vi "Angle Alignment.vi"(9 "IMU Reading":dbl, 10 "Setpoint":dbl) -> (1 "Finished":bool, 2 "output":dbl format="%.2f")   [LabVIEW 2025]
doc: "Heading controller used by the Drive Controller \"Turn Aligning\" mode (structure from Reefscape 2025). Setpoint and IMU Reading are yaw in degrees (rounded to whole degrees). Outside +/- IMU Tolerance it runs a Parallel PID and returns the motor output; inside tolerance output is 0. Default gains: Everybot-tuned P and D (Kp 0.01, Kd 0.0006) plus the Reefscape integral (Ki 0.01), output +/-0.5. Finished is true once the heading is within tolerance AND the robot has settled: Pigeon accelerometer X magnitude < 350 and yaw rate (Pigeon raw gyro Z) magnitude < 5 deg/s."
uses:
  <vilib>/Rock Robotics/WPI/ThirdParty/Phoenix-LabVIEW/Pigeon IMU/CTRE_PigeonIMU_GetBiasedAccelerometer.vi
panel:
  out "Waveform Chart":cluster{i32, i32}(graph)
  in  "IMU Tolerance":dbl=5.0
  in  "IMU":T1={"PID gains IMU"={"proportional gain (Kp)"=0.01, "integral time (Ki)"=0.01, "derivative time (Kd)"=0.0006}, "output range IMU"={"high"=0.5, "low"=-0.5}} {"output range IMU"."low" format="%.2f"; "output range IMU"."high" format="%.2f"; "PID gains IMU"."derivative time (Kd)" format="%.3f"; "PID gains IMU"."integral time (Ki)" format="%.3f"; "PID gains IMU"."proportional gain (Kp)" format="%.3f"}
  in  "FeedFwd Value 2":dbl format="%.2f"
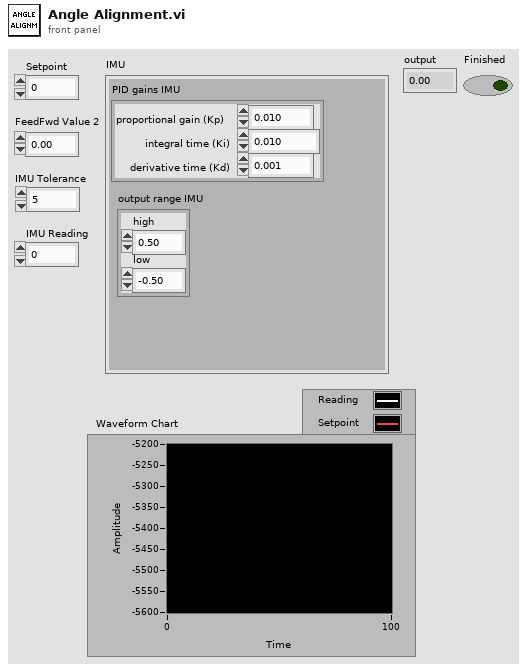
[diagram p1: front panel]
types:
  T1 = cluster{"PID gains IMU":cluster{"proportional gain (Kp)":sgl, "integral time (Ki)":dbl, "derivative time (Kd)":dbl}, "output range IMU":cluster{"high":dbl, "low":dbl}}
  T2 = typedef "CTRE_PigeonIMU_DeviceRef.ctl" = cluster{"DeviceStatus":errorcluster, "Device Number":u8, "Type":T3, "Device ID":u32, "Handle":u64, "UsageFrame":u32, "Library Path":path}
  T3 = typedef "CTRE_PigeonIMU_ConnectionType.ctl" = u32
  T4 = cluster{"X":dbl, "Y":dbl, "Z":dbl, "Magnitude":dbl}
  T5 = cluster{"proportional gain (Kp)":sgl, "integral time (Ki)":dbl, "derivative time (Kd)":dbl}
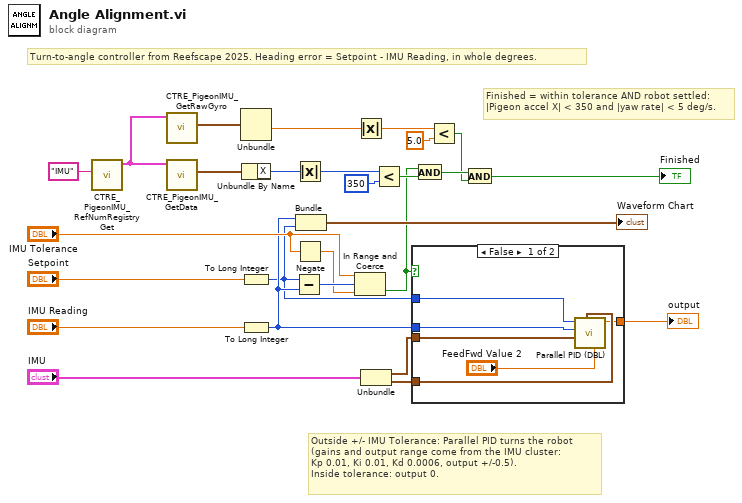
[diagram p0: block diagram]
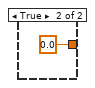
[diagram p2: hidden frame]
diagram:
  # "Outside +/- IMU Tolerance: Parallel PID turns the robot\n(gains and output range come from the IMU cluster:\nKp 0.01, Ki 0.01, Kd 0.0006, output +/-0.5).\nInside tolerance: output 0."
  # "Finished = within tolerance AND robot settled:\n|Pigeon accel X| < 350 and |yaw rate| < 5 deg/s."
  # "Turn-to-angle controller from Reefscape 2025. Heading error = Setpoint - IMU Reading, in whole degrees."
  n1 = call <vilib>:"CTRE_PigeonIMU_RefNumRegistryGet.vi"("refnum name"="IMU") -> ("PigeonIMUDevRef"=w23:T2)  [unwired: 9 in, 1 out]
  n2 = call <vilib>:"CTRE_PigeonIMU_GetRawGyro.vi"("PigeonIMUDevRef"=w23) -> ("Gyro DPS"=w6:T4)  [unwired: 8 in, 2 out]
  n3 = call-poly <vilib>:"CTRE_PigeonIMU_GetData.vi"("PigeonIMUDevRef"=w23) -> ("Biased Accelerometer"=w21:cluster{"X":i16, "Y":i16, "Z":i16, "Norm":i16})  [unwired: 8 in, 2 out]
  n4 = Unbundle(w6) -> ("Z"=w5:dbl)  [unwired: 3 out]
  n5 = To Long Integer(number="Setpoint") -> (32bit integer=w7:i32)
  n6 = To Long Integer(number="IMU Reading") -> (32bit integer=w9:i32)
  n7 = Unbundle By Name(w21) -> ("X"=w18:i16)
  n8 = Subtract(x=w7, y=w9) -> (x-y=w13:i32)
  n9 = Absolute Value(x=w18) -> (abs(x)=w17:i16)
  n10 = Negate(x="IMU Tolerance") -> (-x=w11:dbl)
  n11 = Bundle(w9, w7) -> (→"Waveform Chart":cluster{i32, i32})  [unwired: 1 in]
  n12 = In Range and Coerce(upper limit="IMU Tolerance", x=w13, lower limit=w11) -> (In Range?=w14:bool)  [unwired: 1 out]
  n13 = Absolute Value(x=w5) -> (abs(x)=w4:dbl)
  n14 = Unbundle("IMU") -> ("PID gains IMU"=w27:T5, "output range IMU"=w26:cluster{"high":dbl, "low":dbl})
  n15 = Less?(x=w17, y=i16 350) -> (x < y?=w19:bool)
  n16 = case shown="False" w14 {
    tunnel: w9 -> [w33 _]
    tunnel: [w30 0.0] -> w16
    tunnel: w26 -> [w32 _]
    tunnel: w27 -> [w29 _]
    tunnel: w7 -> [w28 _]
    frame False {
      n17 = call <vilib>:"Parallel PID (DBL).vi"("FeedFwd Value"="FeedFwd Value 2", "output range"=w32, "PID gains"=w29, "process variable"=w33, "setpoint"=w28) -> ("output"=w30:dbl)  [unwired: 3 in, 3 out]
    }
    frame True {
    }
  }
  "output" <- w16
  n18 = And(x=w14, y=w19) -> (x .and. y?=w24:bool)
  n19 = Less?(x=w4, y=5.0) -> (x < y?=w1:bool)
  n20 = And(x=w24, y=w1) -> (x .and. y?=→"Finished":bool)
